vi "ShowHideScrollBar.vi"(8 "error in":errorcluster, 11 "reference":refnum<vi>) -> (0 "error out":errorcluster, 1 "Visible?":bool, 2 "Value":string, 3 "reference out":refnum<vi>)   [LabVIEW 2020]
doc: "This VI compares the number of displayed items in the list with the total number of visible rows and shows/hides the Vertical Scroll Bar as appropriate."
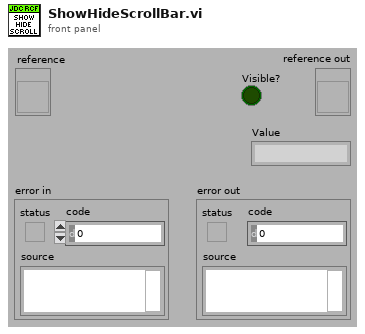
[diagram p1: front panel]
types:
  T1 = typedef "LVNodeAndColumnTypeDef.ctl" = cluster{"Node":string, "Column":i32}
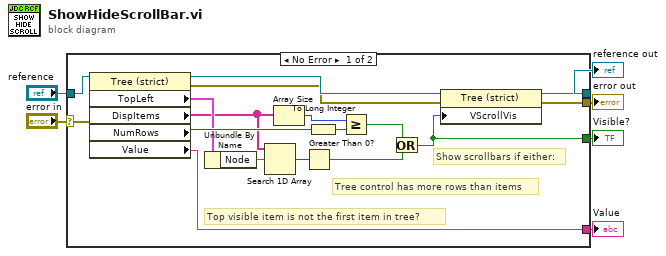
[diagram p0: block diagram]
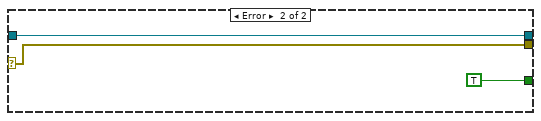
[diagram p2: hidden frame]
diagram:
  n1 = case shown="No Error" "error in" {
    selector: "error in" -> [w15 w26]
    tunnel: "reference" -> [w19 w25]
    tunnel: [w18 _] -> w5
    tunnel: [w17 w25] -> w4
    tunnel: [w16 w26] -> w2
    tunnel: [w7 TRUE] -> w1
    frame No Error {
      # "Show scrollbars if either:"
      # "Tree control has more rows than items"
      # "Top visible item is not the first item in tree?"
      n2 = property class="Tree (strict)"(reference=w19, error in=w15) -> (reference out=w22:refnum<vi>, error out=w21:errorcluster, "TopLeft"=w14:T1, "DispItems"=w13:string[], "NumRows"=w23:u32, "Value"=w18:string)
      n3 = Unbundle By Name(w14) -> ("Node"=w12:string)
      n4 = Search 1D Array(1D array=w13, element=w12) -> (index of element=w10:i32)  [unwired: 1 in]
      n5 = Array Size(array=w13) -> (size(s)=w11:i32)
      n6 = Greater Than 0?(x=w10) -> (x > 0?=w9:bool)
      n7 = To Long Integer(number=w23) -> (32bit integer=w20:i32)
      n8 = Greater Or Equal?(x=w11, y=w20) -> (x >= y?=w8:bool)
      n9 = Or(x=w8, y=w9) -> (x .or. y?=w7:bool)
      n10 = property class="Tree (strict)"(reference=w22, error in=w21, "VScrollVis"=w7) -> (reference out=w17:refnum<vi>, error out=w16:errorcluster)
    }
    frame Error {
    }
  }
  "Value" <- w5
  "reference out" <- w4
  "error out" <- w2
  "Visible?" <- w1
